vi "GetDeviceInfo.vi"(8 "error in":errorcluster, 11 "Device":i32=-1) -> (0 "error out":errorcluster, 3 "CudaDeviceInfo":T1)   [LabVIEW 2020, in "OpenLvVision_OpenCv.lvlib" / "Cuda.lvlib"]
doc: "Retruns information about the device."
uses:
  Cuda.lvlib
  TypeDef/CudaDeviceInfo.ctl
  OpenLvVision_OpenCv.lvlib
  Dlls/OlvOpenCvWrapper.dll
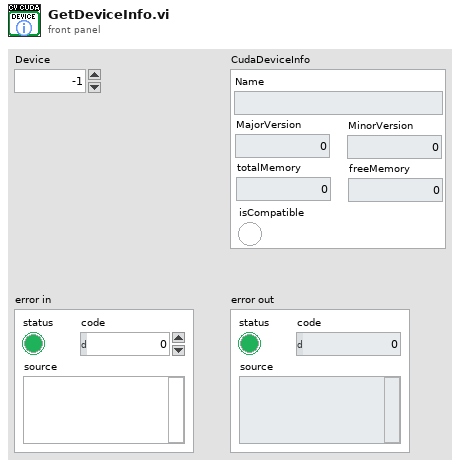
[diagram p1: front panel]
types:
  T1 = typedef "OpenLvVision_OpenCv.lvlib/CudaDeviceInfo.ctl" = cluster{"Name":string, "MajorVersion":i32, "MinorVersion":i32, "totalMemory":i64, "freeMemory":i64, "isCompatible":bool}
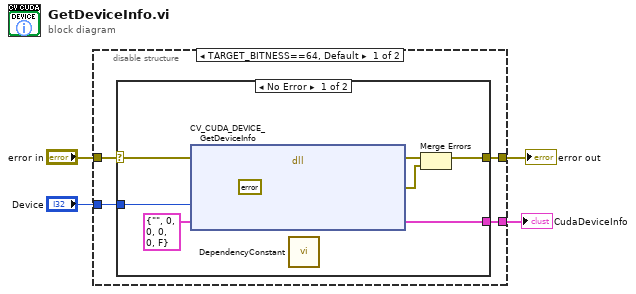
[diagram p0: block diagram]
diagram:
  n1 = disable-structure shown="TARGET_BITNESS==64, Default" {
    disable-tunnel: "error in" -> [w7 w18]
    disable-tunnel: [w8 w18] -> w3
    disable-tunnel: [w6 _] -> w2
    disable-tunnel: "Device" -> [w5 _]
    frame condition #0 (active) {
      n2 = case shown="No Error" w7 {
        selector: w7 -> [w12 w17]
        tunnel: [w13 w17] -> w8
        tunnel: [w11 _] -> w6
        tunnel: w5 -> [w9 _]
        frame No Error {
          n3 = dll-call lib="C:/Users/lukas/Documents/OpenLvVision_OpenCv/SourceCode/LabView/OpenLvVision_OpenCv/Dlls/OlvOpenCvWrapper.dll" fn="CV_CUDA_DEVICE_GetDeviceInfo"(error in=w12, "Error"=errorcluster {"status"=FALSE, "code"=0, "source"=""} ("error out"), "device"=w9, "CudaDeviceInfo"=T1 {"Name"="", "MajorVersion"=0, "MinorVersion"=0, "totalMemory"=0, "freeMemory"=0, "isCompatible"=FALSE}) -> (error out=w16:errorcluster, "Error"=w15:errorcluster, "CudaDeviceInfo"=w11:T1)  [unwired: 4 in, 1 out]
          n4 = call "DependencyConstant.vi"() -> ()  [unwired: 12 in]
          n5 = Merge Errors(w16, w15) -> (w13:errorcluster)
        }
        frame Error {
        }
      }
    }
    frame condition #1 {
    }
  }
  "error out" <- w3
  "CudaDeviceInfo" <- w2
